vi "PicoScopeospaGetValuesOverlapped.vi"(5 "Segment Range":T1 {"toSegmentIndex" format="%.4p"; "fromSegmentIndex" format="%.4p"}, 7 "Buffer and Transfer Settings":T2={"startIndex"=0, "Samples"=1000, "Down Sample Ratio"=1, "Down-Sample Mode"=1} {"Down-Sample Mode" items=["RAW none"=2147483648, "None"=0, "Aggregate"=1, "Decimate"=2, "Average"=4]; "Down Sample Ratio" step=1; "Samples" format="%_6p"}, 8 "error in (no error)":errorcluster, 11 "handle in":i16) -> (0 "error out":errorcluster, 3 "handle out":i16, 4 "Pointer to Overflow":u64[](array[numeric]), 6 "noOfSamples":u64)   [LabVIEW 2010]
doc: "Calls GetValuesOverlapped"
uses:
  psospa.dll
  shared/Segment Range.ctl
  shared/Buffer and Transfer Settings.ctl
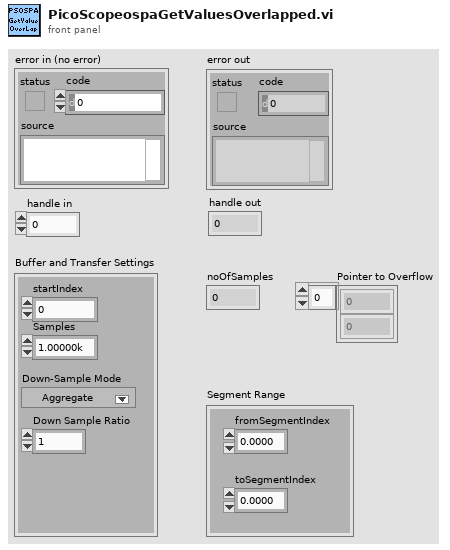
[diagram p1: front panel]
types:
  T1 = typedef "Segment Range.ctl" = cluster{"fromSegmentIndex":u64, "toSegmentIndex":u64}
  T2 = typedef "Buffer and Transfer Settings.ctl" = cluster{"startIndex":u64, "Samples":u64, "Down Sample Ratio":u64, "Down-Sample Mode":u32}
  T3 = cluster{"status":bool, "code":u32, "source":string}
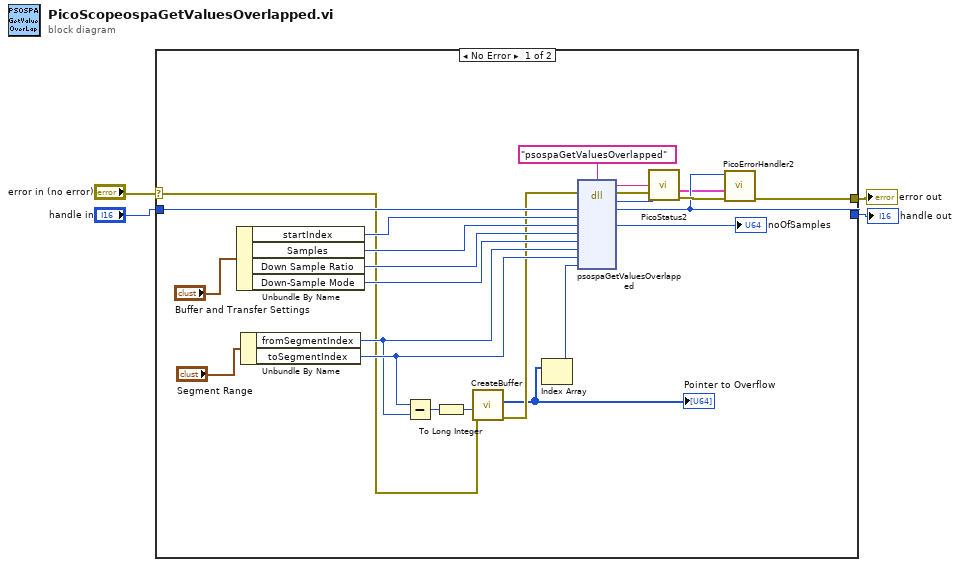
[diagram p0: block diagram]
diagram:
  n1 = case shown="No Error" "error in (no error)" {
    selector: "error in (no error)" -> [w9 w28]
    tunnel: "handle in" -> [w18 w29]
    tunnel: [w16 w29] -> w4
    tunnel: [w17 w28] -> w3
    frame No Error {
      n2 = Unbundle By Name("Buffer and Transfer Settings") -> ("startIndex"=w19:u64, "Samples"=w27:u64, "Down Sample Ratio"=w24:u64, "Down-Sample Mode"=w25:u32)
      n3 = Unbundle By Name("Segment Range") -> ("fromSegmentIndex"=w12:u64, "toSegmentIndex"=w13:u64)
      n4 = Subtract(x=w13, y=w12) -> (x-y=w11:u64)
      n5 = To Long Integer(number=w11) -> (32bit integer=w10:i32)
      n6 = call "CreateBuffer.vi"("error in (no error)"=w9, "Buffer size"=w10) -> ("error out"=w8:errorcluster, "Pointer and BufferSize"=w7:u64[])  [unwired: 8 in]
      "Pointer to Overflow" <- w7
      n7 = Index Array(array=w7) -> (element=w6:u64)  [unwired: 1 in]
      n8 = dll-call lib="psospa.dll" fn="psospaGetValuesOverlapped" ("ps3000.dll:_ps3000_open_unit@0")(error in=w8, "handle"=w18, "startIndex"=w19, "noOfSamples"=w27, "downSampleRatio"=w24, "downSampleRatioMode"=w25, "fromSegmentIndex"=w12, "toSegmentIndex"=w13, "overflow"=w6) -> (error out=w23:errorcluster, "PICO_STATUS"=w22:u32, "handle"=w16:i16, "noOfSamples"=→"noOfSamples":u64)  [unwired: 8 in, 1 out]
      n9 = call "PicoStatus2.vi"("PICO source"="psospaGetValuesOverlapped" ("source"), "Error in"=w23, "PICO STATUS"=w22) -> ("error out"=w26:errorcluster, "PICO_STATUS out"=w5:T3)  [unwired: 5 in]
      n10 = call "PicoErrorHandler2.vi"("error in (no error)"=w26, "PICO_STATUS in"=w5, "handle In"=w16) -> ("error out"=w17:errorcluster)  [unwired: 8 in]
    }
    frame Error {
    }
  }
  "error out" <- w3
  "handle out" <- w4
